vi "VIH HelpGen - HTML - Encode string to HTML format (pass tags).vi"(8 "HTML Tagset allowed":T1(ring), 10 "Reject CR (F)":bool, 11 "string":string) -> (3 "HTML string":string)   [LabVIEW 2014]
doc: "::: VI Helpeks :::\nCopyright (c) 2000-2026 Konstantin Shifershteyn. All rights reserved."
panel:
  # "VI Helpeks\nCopyright (c) 2012-2026 Konstantin Shifershteyn"
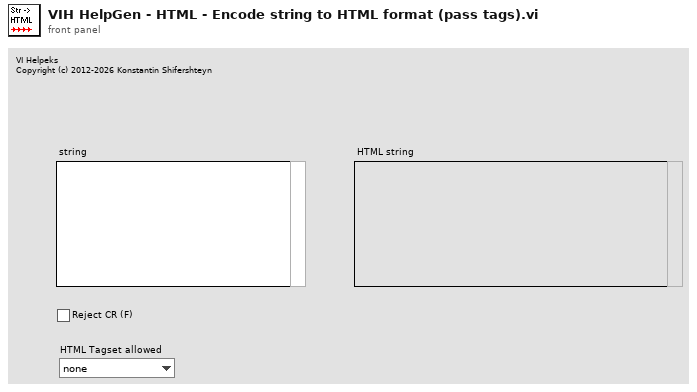
[diagram p1: front panel]
types:
  T1 = enum16{"none", "LV description", "VH minimum", "VH extended"}
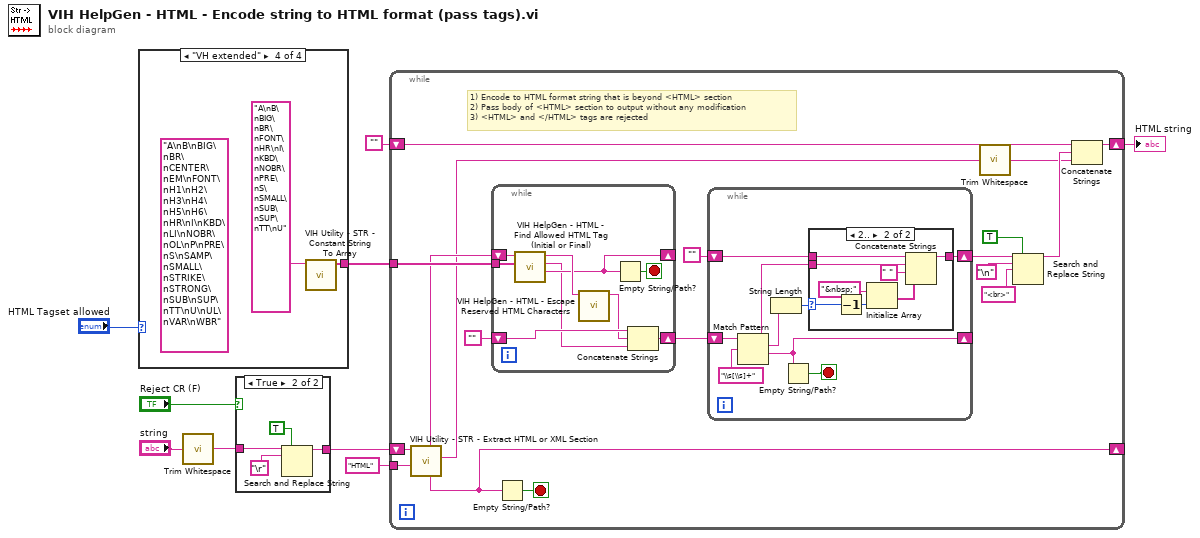
[diagram p0: block diagram]
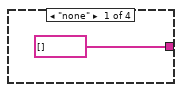
[diagram p2: hidden frame]
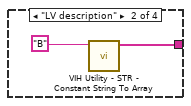
[diagram p3: hidden frame]
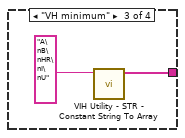
[diagram p4: hidden frame]
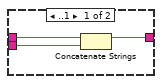
[diagram p5: hidden frame]
diagram:
  n1 = case shown="\"VH extended\"" "HTML Tagset allowed" {
    tunnel: [string[] [] ("Array out") w12 w14 w16] -> w1
    frame "none" {
    }
    frame "LV description" {
      n2 = call "VIH Utility - STR - Constant String To Array.vi"("String in"="B") -> ("Array out"=w12:string[])  [unwired: 10 in]
    }
    frame "VH minimum" {
      n3 = call "VIH Utility - STR - Constant String To Array.vi"("String in"="A\nB\nHR\nI\nU") -> ("Array out"=w14:string[])  [unwired: 10 in]
    }
    frame "VH extended" {
      (unwired) "A\nB\nBIG\nBR\nCENTER\nEM\nFONT\nH1\nH2\nH3\nH4\nH5\nH6\nHR\nI\nKBD\nLI\nNOBR\nOL\nP\nPRE\nS\nSAMP\nSMALL\nSTRIKE\nSTRONG\nSUB\nSUP\nTT\nU\nUL\nVAR\nWBR" ("String in")
      n4 = call "VIH Utility - STR - Constant String To Array.vi"("String in"="A\nB\nBIG\nBR\nFONT\nHR\nI\nKBD\nNOBR\nPRE\nS\nSMALL\nSUB\nSUP\nTT\nU") -> ("Array out"=w16:string[])  [unwired: 10 in]
    }
  }
  n5 = call <vilib>:"Trim Whitespace.vi"("string"="string") -> ("trimmed string"=w8:string)  [unwired: 1 in]
  n6 = case shown="True" "Reject CR (F)" {
    tunnel: w8 -> [w17 w21]
    tunnel: [w17 w20] -> w6
    frame False {
    }
    frame True {
      n7 = Search and Replace String(replace all?=TRUE, input string=w21, search string="\r") -> (result string=w20:string)  [unwired: 5 in, 3 out]
    }
  }
  n8 = while {
    tunnel: w1 -> [w32]
    shift-right: [w30] -> _
    shift-left: w6 -> [w31]
    tunnel: "HTML" -> [w27]
    shift-right: [w25] -> w3
    shift-left: "" -> [w26]
    stop <- w29 stop-if-true
    # "1) Encode to HTML format string that is beyond <HTML> section\n2) Pass body of <HTML> section to output without any modification\n3) <HTML> and </HTML> tags are rejected"
    n9 = call "VIH Utility - STR - Extract HTML or XML Section.vi"("Section name"=w27, "HTML in"=w31) -> ("body"=w24:string, "after"=w30:string, "before"=w28:string)  [unwired: 5 in, 2 out]
    n10 = while {
      shift-right: [w41] -> _
      shift-left: w28 -> [w44]
      shift-right: [w48] -> w33
      shift-left: "" -> [w47]
      tunnel: w32 -> [w43]
      stop <- w46 stop-if-true
      n11 = call "VIH HelpGen - HTML - Find Allowed HTML Tag (Initial or Final).vi"("Tags (upper case)"=w43, "String"=w44) -> ("After"=w41:string, "Match"=w40:string, "Before"=w42:string)  [unwired: 6 in, 1 out]
      n12 = call "VIH HelpGen - HTML - Escape Reserved HTML Characters.vi"("string"=w42) -> ("HTML string"=w45:string)  [unwired: 10 in]
      n13 = Empty String/Path?(string/path=w41) -> (empty?=w46:bool)
      n14 = Concatenate Strings(w47, w45, w40) -> (w48:string)
    }
    n15 = Empty String/Path?(string/path=w30) -> (empty?=w29:bool)
    n16 = while {
      shift-right: [w55] -> _
      shift-left: w33 -> [w57]
      shift-right: [w52] -> w38
      shift-left: "" -> [w51]
      stop <- w54 stop-if-true
      n17 = Match Pattern(string=w57, regular expression="\\s[\\s]+") -> (before substring=w50:string, match substring=w53:string, after substring=w55:string)  [unwired: 1 in, 1 out]
      n18 = String Length(string=w53) -> (length=w49:i32)
      n19 = Empty String/Path?(string/path=w55) -> (empty?=w54:bool)
      n20 = case shown="2.." w49 {
        selector: w49 -> [_ w62]
        tunnel: [w58 w65] -> w52
        tunnel: w51 -> [w60 w64]
        tunnel: w50 -> [w59 w63]
        frame ..1 {
          n21 = Concatenate Strings(w60, w59) -> (w58:string)
        }
        frame 2.. {
          n22 = Decrement(x=w62) -> (x-1=w68:i32)
          n23 = Initialize Array("&nbsp;", w68) -> (w66:string[])
          n24 = Concatenate Strings(w64, w63, " " ("string"), w66) -> (w65:string)
        }
      }
    }
    n25 = call <vilib>:"Trim Whitespace.vi"("string"=w24) -> ("trimmed string"=w22:string)  [unwired: 1 in]
    n26 = Search and Replace String(replace all?=TRUE, input string=w38, search string="\n", replace string="<br>") -> (result string=w23:string)  [unwired: 4 in, 3 out]
    n27 = Concatenate Strings(w26, w23, w22) -> (w25:string)
  }
  "HTML string" <- w3
